vi "Test Start and Stop Entry.vi"(8 "error in":errorcluster, 10 "Work Folder":path, 11 "Test Data Folder":path) -> (0 "error out":errorcluster, 2 "Report":string, 3 "Passed":bool)   [LabVIEW 2026]
doc: "Tests Start Entry.vi and Stop Entry.vi on a copy of the schema-v2 sample data. Entries start on 2026-01-15 10:00 UTC, so they go to 2026-01.ini, a month file the samples do not have. Checks: Start Entry with an empty Task ID returns error 5101 and writes nothing; Start Entry gives the new entry an ID and saves it running (End Time = \"\") with the project name label; Stop Entry writes the End Time into the file and returns a cleared Active Entry out; Stop Entry with an empty Active Entry changes nothing.\n\nInputs: Test Data Folder; Work Folder; error in. Outputs: Passed; Report; error out.\n\nGenerated by: Claude"
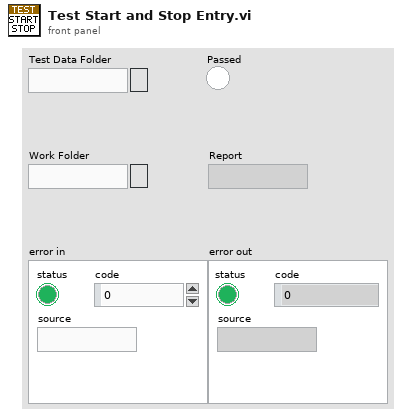
[diagram p1: front panel]
types:
  T1 = typedef "Time Entry.ctl" = cluster{"ID":string, "Project ID":string, "Task ID":string, "Start Time":timestamp, "End Time":timestamp, "Description":string}
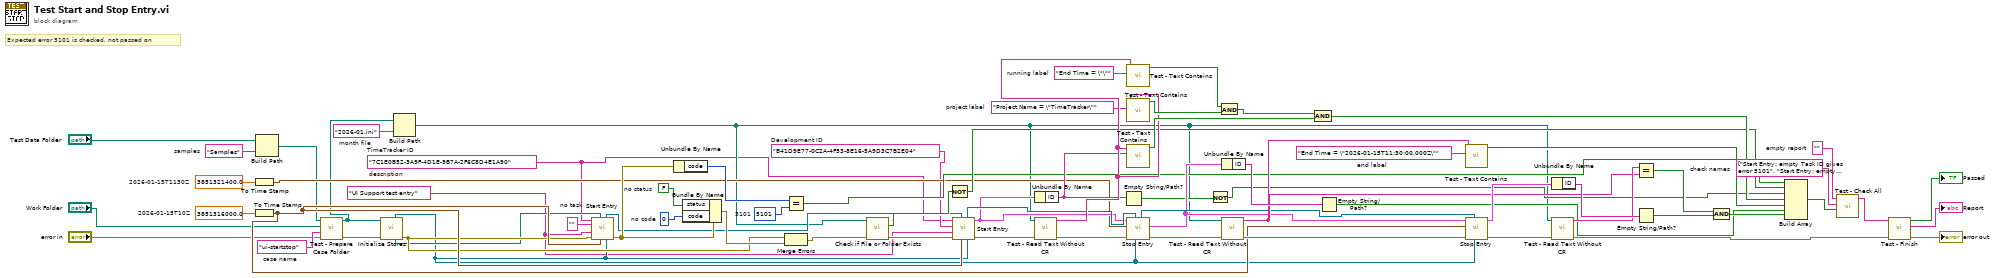
[diagram p0: block diagram]
diagram:
  w23 = string[] ["Start Entry: empty Task ID gives error 5101", "Start Entry: empty Task ID writes nothing", "Start Entry: the new entry has an ID", "Start Entry: saved running (End Time empty) with the project name label", "Stop Entry: the file holds the End Time", "Stop Entry: Active Entry out is cleared", "Stop Entry: an empty Active Entry changes nothing"]  # check names
  w22 = "End Time = \"2026-01-15T11:30:00.000Z\""  # end label
  w21 = "Project Name = \"TimeTracker\""  # project label
  w20 = "End Time = \"\""  # running label
  w19 = 0  # no code
  w18 = FALSE  # no status
  w17 = 5101  # 5101
  w16 = 3851321400.0  # 2026-01-15T1130Z
  w15 = 3851316000.0  # 2026-01-15T10Z
  w14 = "UI Support test entry"  # description
  w13 = ""  # no task
  w12 = "B41D9E77-0C2A-4F53-8E16-5A9D3C7B2E04"  # Development ID
  w11 = "7C1E0B52-3A9F-4D1E-9B7A-2F6C8D4E1A90"  # TimeTracker ID
  w10 = "2026-01.ini"  # month file
  w9 = ""  # empty report
  w8 = "ui-startstop"  # case name
  w7 = "Samples"  # samples
  # "Expected error 5101 is checked, not passed on"
  n1 = To Time Stamp(1:w16) -> (0:w32:timestamp)
  n2 = To Time Stamp(1:w15) -> (0:w31:timestamp)
  n3 = Build Path(base path="Test Data Folder", name or relative path=w7) -> (appended path=w24:path)
  n4 = call "Test - Prepare Case Folder.vi"("error in (no error)"="error in", "Case Name"=w8, "Work Folder"="Work Folder", "Source Folder"=w24) -> ("error out"=w26:errorcluster, "Case Folder"=w25:path)  [unwired: 6 in]
  n5 = call "Initialize Stores.vi"("error in"=w26, "Data Folder"=w25) -> ("error out"=w30:errorcluster, "Time Entry Store out"=w29:refnum<class "Time Entry Store.lvclass">, "Project Store out"=w28:refnum<class "Project Store.lvclass">)  [unwired: 5 in, 2 out]
  n6 = Build Path(base path=w25, name or relative path=w10) -> (appended path=w27:path)
  n7 = call "Start Entry.vi"("Project Store in"=w28, "Start Time"=w31, "Time Entry Store in"=w29, "error in"=w30, "Description"=w14, "Task ID"=w13, "Project ID"=w11) -> ("error out"=w34:errorcluster, "Time Entry Store out"=w33:refnum<class "Time Entry Store.lvclass">)  [unwired: 2 in, 1 out]
  n8 = Unbundle By Name(w34) -> ("code"=w35:i32)
  n9 = Bundle By Name(cluster=w34, "status"=w18, "code"=w19) -> (w37:errorcluster)
  n10 = Equal?(x=w35, y=w17) -> (x = y?=w36:bool)
  n11 = Merge Errors(w30, w37) -> (w38:errorcluster)
  n12 = call <vilib>:"Check if File or Folder Exists.vi"("error in (no error)"=w38, "path"=w27) -> ("error out"=w40:errorcluster, "file or folder exists?"=w39:bool)  [unwired: 7 in, 1 out]
  n13 = Not(x=w39) -> (.not. x?=w41:bool)
  n14 = call "Start Entry.vi"("Project Store in"=w28, "Start Time"=w31, "Time Entry Store in"=w33, "error in"=w40, "Description"=w14, "Task ID"=w12, "Project ID"=w11) -> ("error out"=w44:errorcluster, "New Entry"=w42:T1, "Time Entry Store out"=w43:refnum<class "Time Entry Store.lvclass">)  [unwired: 2 in]
  n15 = Unbundle By Name(w42) -> ("ID"=w45:string)
  n16 = call "Test - Read Text Without CR.vi"("error in (no error)"=w44, "File"=w27) -> ("error out"=w49:errorcluster, "Text"=w48:string)  [unwired: 8 in]
  n17 = Empty String/Path?(string/path=w45) -> (empty?=w46:bool)
  n18 = call "Test - Text Contains.vi"("Search Text"=w20, "Text"=w48) -> ("Contains?"=w50:bool)  [unwired: 8 in, 1 out]
  n19 = call "Test - Text Contains.vi"("Search Text"=w21, "Text"=w48) -> ("Contains?"=w51:bool)  [unwired: 8 in, 1 out]
  n20 = call "Test - Text Contains.vi"("Search Text"=w45, "Text"=w48) -> ("Contains?"=w52:bool)  [unwired: 8 in, 1 out]
  n21 = call "Stop Entry.vi"("Project Store in"=w28, "Time Entry Store in"=w43, "error in"=w49, "End Time"=w32, "Active Entry"=w42) -> ("error out"=w57:errorcluster, "Active Entry out"=w55:T1, "Time Entry Store out"=w56:refnum<class "Time Entry Store.lvclass">)  [unwired: 3 in, 1 out]
  n22 = Not(x=w46) -> (.not. x?=w47:bool)
  n23 = And(x=w50, y=w51) -> (x .and. y?=w53:bool)
  n24 = Unbundle By Name(w55) -> ("ID"=w61:string)
  n25 = call "Test - Read Text Without CR.vi"("error in (no error)"=w57, "File"=w27) -> ("error out"=w59:errorcluster, "Text"=w58:string)  [unwired: 8 in]
  n26 = And(x=w53, y=w52) -> (x .and. y?=w54:bool)
  n27 = Empty String/Path?(string/path=w61) -> (empty?=w62:bool)
  n28 = call "Test - Text Contains.vi"("Search Text"=w22, "Text"=w58) -> ("Contains?"=w60:bool)  [unwired: 8 in, 1 out]
  n29 = call "Stop Entry.vi"("Project Store in"=w28, "Time Entry Store in"=w56, "error in"=w59, "End Time"=w31, "Active Entry"=w55) -> ("error out"=w64:errorcluster, "Stopped Entry"=w63:T1)  [unwired: 3 in, 2 out]
  n30 = Unbundle By Name(w63) -> ("ID"=w68:string)
  n31 = call "Test - Read Text Without CR.vi"("error in (no error)"=w64, "File"=w27) -> ("error out"=w66:errorcluster, "Text"=w65:string)  [unwired: 8 in]
  n32 = Equal?(x=w65, y=w58) -> (x = y?=w67:bool)
  n33 = Empty String/Path?(string/path=w68) -> (empty?=w69:bool)
  n34 = And(x=w67, y=w69) -> (x .and. y?=w70:bool)
  n35 = Build Array(w36, w41, w47, w54, w60, w62, w70) -> (w71:bool[])
  n36 = call "Test - Check All.vi"("Conditions"=w71, "Check Names"=w23, "Report in"=w9) -> ("Report out"=w72:string)  [unwired: 7 in, 1 out]
  n37 = call "Test - Finish.vi"("error in (no error)"=w66, "Report"=w72) -> ("error out"=→"error out":errorcluster, "Report out"=→"Report":string, "Passed"=→"Passed":bool)  [unwired: 7 in]
